vi "Benchmark_GetName.vi"() -> ()   [LabVIEW 2013]
uses:
  <vilib>/Utility/VariantDataType/SetTypeInfo.vi
  <vilib>/Utility/VariantDataType/GetTypeInfo.vi
  source/Variant/OpenVariant.lvlib
panel:
  out "Array":string[](array[string])
  out "Waveform Chart":dbl(graph)
  out "execution time per call":dbl
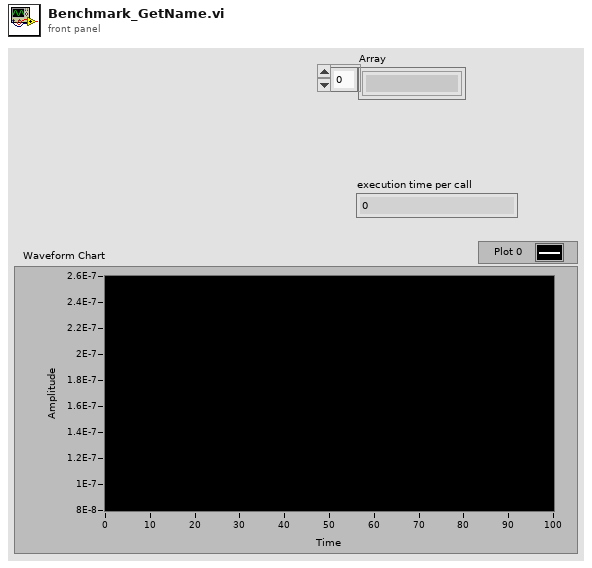
[diagram p1: front panel]
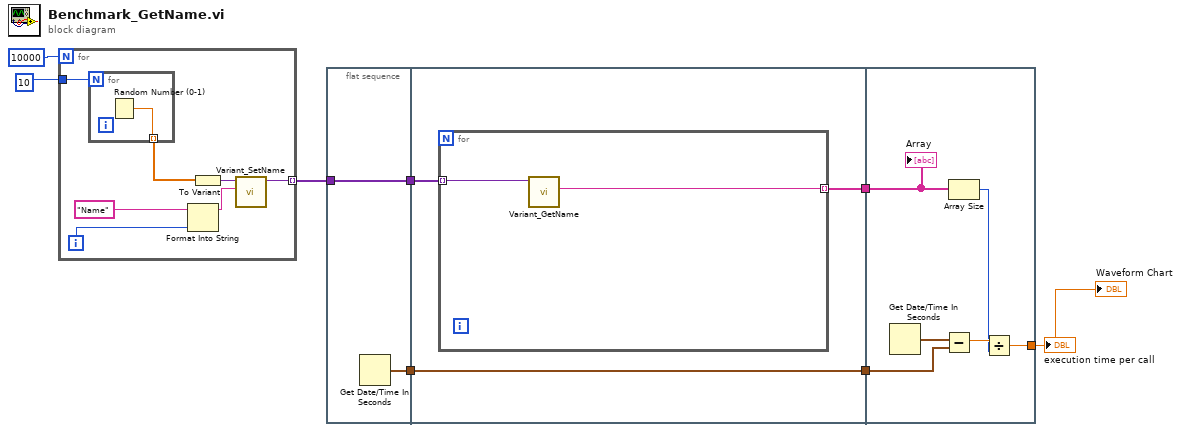
[diagram p0: block diagram]
diagram:
  n1 = for {
    N: 10000 -> [_]
    tunnel: [w12] -> w7 mode=indexing
    tunnel: 10 -> [w9]
    i -> [w11]
    n2 = for {
      N: w9 -> [_]
      tunnel: [w16] -> w10 mode=indexing
      n3 = Random Number (0-1)() -> (number: 0 to 1=w16:dbl)
    }
    n4 = Format Into String(initial string="Name", w11) -> (resulting string=w13:string)  [unwired: 2 in, 1 out]
    n5 = To Variant(anything=w10) -> (Variant=w14:variant)
    n6 = call "Variant_SetName.vi"("Name"=w13, "Variant"=w14) -> ("Named Variant"=w12:variant)  [unwired: 9 in]
  }
  n7 = flat-sequence {
    tunnel: w7 -> [w18]
    tunnel: [w18] -> w6
    tunnel: [w17] -> w4
    tunnel: w6 -> [w21]
    tunnel: [w20] -> w5
    tunnel: w4 -> [w20]
    tunnel: [w19] -> w2
    tunnel: w5 -> [w28]
    tunnel: [w25] -> w3
    tunnel: w2 -> [w24]
    frame #0 {
      n8 = Get Date/Time In Seconds() -> (seconds since 1Jan1904=w17:timestamp)
    }
    frame #1 {
      n9 = for {
        tunnel: w21 -> [w23] mode=indexing
        tunnel: [w22] -> w19 mode=indexing
        n10 = call "Variant_GetName.vi"("Variant"=w23) -> ("Name"=w22:string)  [unwired: 8 in, 2 out]
      }
    }
    frame #2 {
      n11 = Get Date/Time In Seconds() -> (seconds since 1Jan1904=w29:timestamp)
      n12 = Subtract(x=w29, y=w28) -> (x-y=w27:dbl)
      n13 = Array Size(array=w24) -> (size(s)=w26:i32)
      n14 = Divide(x=w27, y=w26) -> (x/y=w25:dbl)
      "Array" <- w24
    }
  }
  "execution time per call" <- w3
  "Waveform Chart" <- w3
